vi "Test Process within Nested App Log Info Message.vi"(8 "error in (no error)":errorcluster, 11 "Test Case In":refnum<class "Logger Test.lvclass">) -> (0 "error out":errorcluster, 3 "Test Case Out":refnum<class "Logger Test.lvclass">)   [LabVIEW 2020, in "Logger Test.lvclass"]
uses:
  Logger Test.lvclass
  C:/Program Files (x86)/National Instruments/LabVIEW 2020/vi.lib/Astemes/LUnit/Test Case.lvclass
  source/Framework Test Suite/Mock Log Handler/Mock Log Handler.lvclass
  C:/git/astemes-triarc-framework/source/Framework/Logging/Logging.lvclass
  source/Framework Test Suite/Mock Process/Mock Process.lvclass
  C:/git/astemes-triarc-framework/source/Framework/Process/Process.lvclass
  source/Framework/Application/Application.lvclass
  source/Framework/Process/Process.lvclass/Process.ctl
  source/Framework/Application/Application.lvclass/Application.ctl
  <vilib>/Astemes/LUnit/Test Case.lvclass/Test Case.ctl
  9c4a66fc-af29-4a58-8a71-606aefca4567.vi
  ff660fc9-a87e-4241-bf4f-74109907e361.vi
  4b535133-13cd-4873-93c4-223ebd3dba1f.vi
  source/Framework/Application/Private/Add Process to Map.vi
  source/Framework/Application/Private/Throw Error If Process Already in App.vi
  source/Framework/Process/Protected/Messaging/Send Message.vi
  source/Framework/Process/Public/Lifecycle/Get Lifecycle State.vi
  source/Framework/Process/Protected/SubVIs/Set Context.vi
  source/Framework/Process/Private/SubVIs/Wait for finish.vi
  source/Framework/Process/Private/SubVIs/Set Lifecycle State.vi
  <vilib>/Astemes/LUnit/Append Pass Result.vi
  <vilib>/Astemes/LUnit/Append Fail Result.vi
  <vilib>/Astemes/LUnit/Describe Comparison.vi
  <vilib>/Astemes/LUnit/Compare Variants.vi
  source/Framework/Application/Public/Get Process.vi
  source/Framework/Process/Private/SubVIs/Handle Debug Data.vi
  <vilib>/Astemes/LUnit/Variant to string.vi
  source/Framework/Application/Private/Retrieve Process from App.vi
  source/Framework/Application/Private/Parse Process Name.vi
  source/Framework/Application/Private/Get Process from Map.vi
  source/Framework/Logging/Log Debug.vi
  <vilib>/AdvancedString/1D String Array to Delimited String.vi
  <vilib>/Utility/High Resolution Relative Seconds.vi
  source/Framework/Process/Protected/Messaging/Request Message.vi
  <vilib>/AdvancedString/Delimited String to 1D String Array.vi
  source/Framework/Process/Private/SubVIs/Enqueue Request Message.vi
  source/Framework/Process/Process.lvclass
  <vilib>/Utility/error.llb/Error Cluster From Error Code.vi
  source/Framework/Process/Public/Read Name.vi
  source/Framework/Process/Private/SubVIs/Wait for Response Message.vi
  <vilib>/Utility/Data Type/Get Type Information.vi
  <vilib>/Utility/LVClass/Get LV Class Name.vi
  source/Framework/Logging/Logging.lvclass
  Logger Test.lvclass/Logger Test.ctl
  source/Framework Test Suite/Support/Test Support.lvlib
  C:/git/astemes-triarc-framework/source/Framework/Base/Base.lvclass
  C:/git/astemes-triarc-framework/source/Framework/Error Handler Interface/Error Handler Interface.lvclass
  C:/git/astemes-triarc-framework/source/Framework/Application/Application.lvclass
  C:/git/astemes-triarc-framework/source/Framework/Async Handler/Async Handler.lvclass
  C:/git/astemes-triarc-framework/source/Framework/Configuration File/Configuration File.lvclass
  C:/git/astemes-triarc-framework/source/Framework/Configuration/Configuration.lvclass
  C:/git/astemes-triarc-framework/source/Framework Test Suite/Mock Process/Mock Process.lvclass
  C:/git/astemes-triarc-framework/source/Framework/Helper Loop/Helper Loop.lvclass
  C:/git/astemes-triarc-framework/source/Framework Test Suite/Mock Log Handler/Mock Log Handler.lvclass
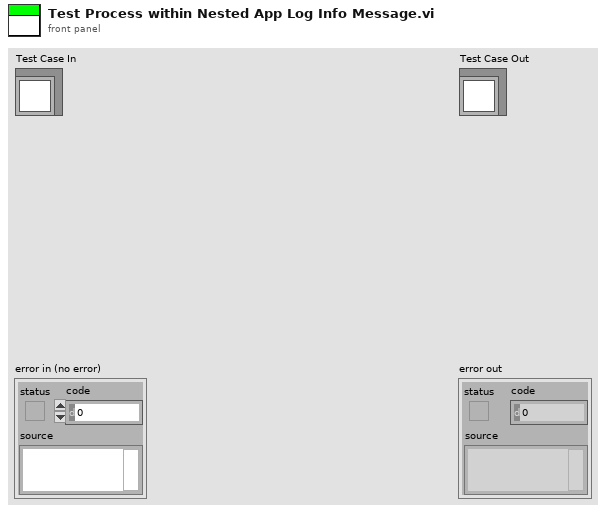
[diagram p1: front panel]
types:
  T1 = typedef "Mock Log Handler.lvclass/Log Entry.ctl" = cluster{"Level":string, "Source":string, "Message":string}
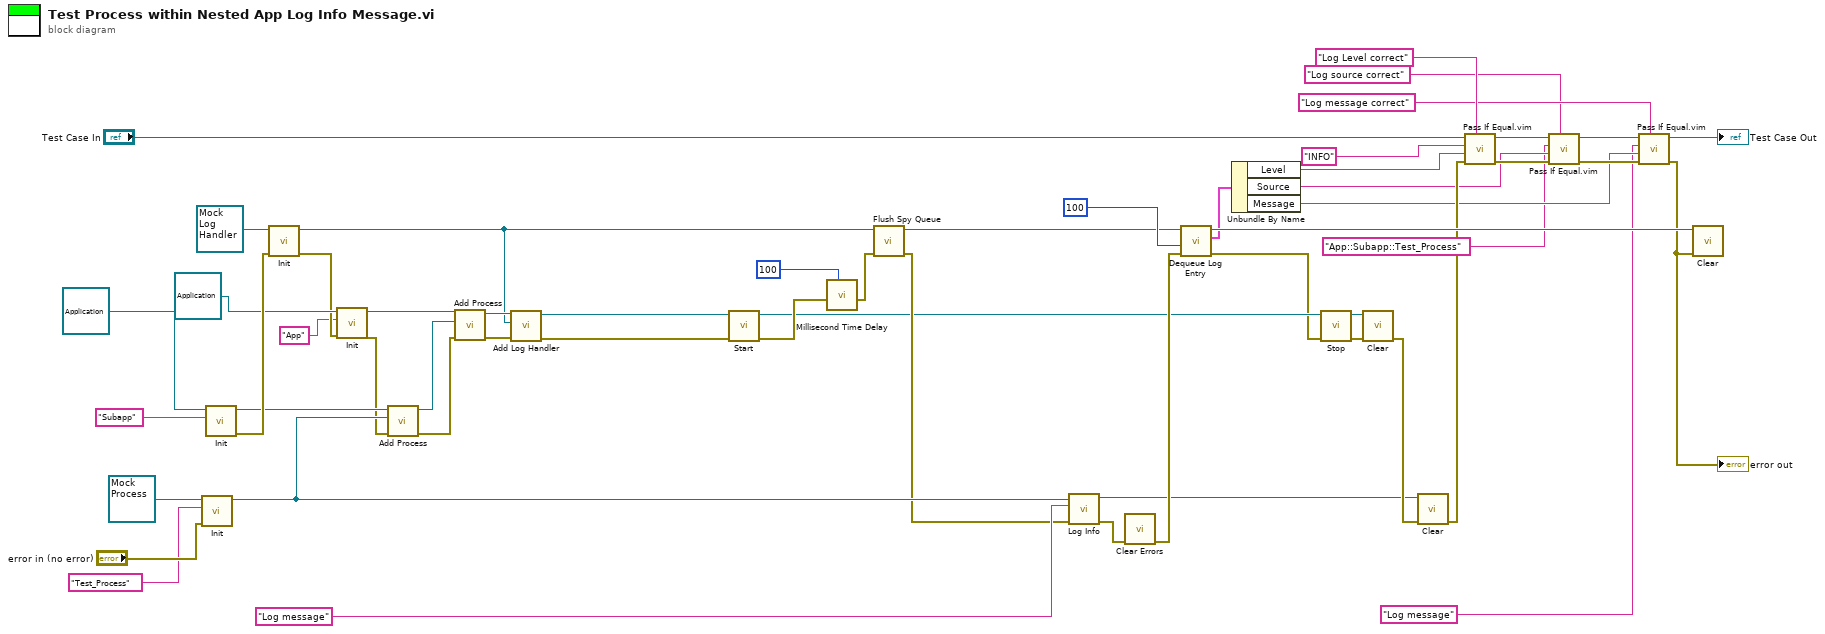
[diagram p0: block diagram]
diagram:
  n1 = call-dynamic "Init.vi"("error in (no error)"="error in (no error)", "Name"="Test_Process", "Mock Process In"=refnum<class "Mock Process.lvclass"> refnum) -> ("Mock Process Out"=w19:refnum<class "Mock Process.lvclass">)  [unwired: 7 in, 1 out]
  n2 = call-dynamic "Init.vi"("Name"="Subapp", "Process In"=refnum<class "Application.lvclass"> refnum ("Application.lvclass")) -> ("error out"=w50:errorcluster, "Process Out"=w11:refnum<class "Application.lvclass">)  [unwired: 8 in]
  n3 = call-dynamic "Init.vi"("error in (no error)"=w50, "Mock Log Handler In"=refnum<class "Mock Log Handler.lvclass"> refnum ("Mock Log Handler.lvclass")) -> ("error out"=w16:errorcluster, "Mock Log Handler Out"=w12:refnum<class "Mock Log Handler.lvclass">)  [unwired: 8 in]
  n4 = call-dynamic "Init.vi"("error in (no error)"=w16, "Name"="App", "Process In"=refnum<class "Application.lvclass"> refnum ("Application.lvclass")) -> ("error out"=w9:errorcluster, "Process Out"=w15:refnum<class "Application.lvclass">)  [unwired: 7 in]
  n5 = call "Add Process.vi"("error in (no error)"=w9, "Process"=w19, "Application In"=w11) -> ("error out"=w8:errorcluster, "Application Out"=w10:refnum<class "Application.lvclass">)  [unwired: 7 in]
  n6 = call "Add Process.vi"("error in (no error)"=w8, "Process"=w10, "Application In"=w15) -> ("error out"=w13:errorcluster, "Application Out"=w14:refnum<class "Application.lvclass">)  [unwired: 7 in]
  n7 = call "Add Log Handler.vi"("error in (no error)"=w13, "Log Handler"=w12, "Process In"=w14) -> ("error out"=w7:errorcluster, "Process Out"=w5:refnum<class "Application.lvclass">)  [unwired: 7 in]
  n8 = call "Start.vi"("error in (no error)"=w7, "Process In"=w5) -> ("error out"=w6:errorcluster, "Process Out"=w4:refnum<class "Application.lvclass">)  [unwired: 7 in, 1 out]
  n9 = call "Millisecond Time Delay.vi"("milliseconds to wait"=u32 100, "error in (no error)"=w6) -> ("error out"=w21:errorcluster)  [unwired: 7 in]
  n10 = call "Flush Spy Queue.vi"("error in (no error)"=w21, "Mock Log Handler in"=w12) -> ("error out"=w18:errorcluster, "Mock Log Handler out"=w22:refnum<class "Mock Log Handler.lvclass">)  [unwired: 7 in, 1 out]
  n11 = call "Log Info.vi"("error in (no error)"=w18, "Message"="Log message", "Logging In"=w19) -> ("error out"=w34:errorcluster, "Logging Out"=w24:refnum<class "Mock Process.lvclass">)  [unwired: 7 in]
  n12 = call <vilib>:"Clear Errors.vi"("error in (no error)"=w34) -> ("error out"=w33:errorcluster)  [unwired: 5 in, 1 out]
  n13 = call "Dequeue Log Entry.vi"("error in (no error)"=w33, "timeout in ms (-1)"=100, "Mock Log Handler in"=w22) -> ("error out"=w1:errorcluster, "Entry"=w47:T1, "Mock Log Handler out"=w49:refnum<class "Mock Log Handler.lvclass">)  [unwired: 5 in, 1 out]
  n14 = Unbundle By Name(w47) -> ("Level"=w46:string, "Source"=w37:string, "Message"=w36:string)
  n15 = call "Stop.vi"("error in (no error)"=w1, "Process In"=w4) -> ("error out"=w26:errorcluster, "Process Out"=w25:refnum<class "Application.lvclass">)  [unwired: 7 in, 1 out]
  n16 = call-dynamic "Clear.vi"("error in (no error)"=w26, "Application In"=w25) -> ("error out"=w52:errorcluster)  [unwired: 9 in]
  n17 = call-dynamic "Clear.vi"("error in (no error)"=w52, "Mock Process In"=w24) -> ("error out"=w40:errorcluster)  [unwired: 9 in]
  n18 = call "Pass If Equal.vim"("Description"="Log Level correct", "error in (no error)"=w40, "Actual"=w46, "Expected"="INFO", "LUnit Test Case In"="Test Case In") -> ("error out"=w42:errorcluster, "LUnit Test Case Out"=w54:refnum<class "Logger Test.lvclass">)  [unwired: 5 in]
  n19 = call "Pass If Equal.vim"("Description"="Log source correct", "error in (no error)"=w42, "Actual"=w37, "Expected"="App::Subapp::Test_Process" ("Name"), "LUnit Test Case In"=w54) -> ("error out"=w41:errorcluster, "LUnit Test Case Out"=w44:refnum<class "Logger Test.lvclass">)  [unwired: 5 in]
  n20 = call "Pass If Equal.vim"("Description"="Log message correct", "error in (no error)"=w41, "Actual"=w36, "Expected"="Log message" ("Message"), "LUnit Test Case In"=w44) -> ("error out"=w2:errorcluster, "LUnit Test Case Out"=→"Test Case Out":refnum<class "Logger Test.lvclass">)  [unwired: 5 in]
  "error out" <- w2
  n21 = call-dynamic "Clear.vi"("error in (no error)"=w2, "Mock Log Handler In"=w49) -> ()  [unwired: 9 in, 1 out]
